vi "Event handler-Z Setup.vi"(8 "error in (no error)":errorcluster, 9 "Obtain Z Stop":bool, 11 "Obtain Z Start":bool) -> (0 "error out":errorcluster)   [LabVIEW 2020]
uses:
  Typedefs/Read Write Enum.ctl
  Global Variables/gl_UI Ctrl Refs.vi
  Global Variables/General Globals.vi
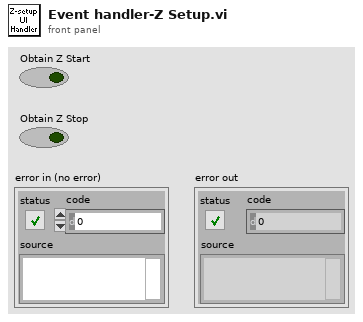
[diagram p1: front panel]
types:
  T1 = typedef "Read Write Enum.ctl" = enum16{"Read", "Write"}
  T2 = typedef "UI ctrl refs cluster.ctl" = cluster{"Top level VI path":path, "Top level VI ref":refnum<vi>, "User menu ref":refnum<k9>, "Sub Panel control":refnum<vi>, "Imaging Param Tab":refnum<vi>, "Occurrence-Start drivers":refnum<k4>, "Occurrence-Speed logging initialised":refnum<k4>, "Occurrence-XYZ stage initialised":refnum<k4>, "Exit button":refnum<vi>, "Status ind":refnum<vi>, "Set as origin":refnum<vi>, "Speed Logging":refnum<vi>, "Time Lapse":refnum<vi>, "Live Imaging":refnum<vi>, "AOL Z Stack":refnum<vi>, "Motor Z Stack":refnum<vi>, "Funct Acq button":refnum<vi>, "Hard Shutter":refnum<vi>, "Virtual Shutter":refnum<vi>, "Laser Power":refnum<vi>, "AOL Mode":refnum<vi>, "Frame Size":refnum<vi>, "Field of View":refnum<vi>, "Dwell Time":refnum<vi>, "Zoom":refnum<vi>, "AOL Z":refnum<vi>, "Objective":refnum<vi>, "Axis":refnum<vi>, "Paths & Names":refnum<vi>, "Experiment folder path (ind.)":refnum<vi>, "Last State (Ind.)":refnum<vi>, "Averages":refnum<vi>, "Angle (degrees)":refnum<vi>, "X centre":refnum<vi>, "Y centre":refnum<vi>, "Plane Mode":refnum<vi>, "# Planes":refnum<vi>, "Z Start":refnum<vi>, "Z Stop":refnum<vi>, "Z Step":refnum<vi>, "PMT 1":refnum<vi>, "PMT 2":refnum<vi>, "Stage XYZ Position":refnum<vi>, "Pockels@Z Start":refnum<vi>, "Pockels@Z Stop":refnum<vi>, "Obtain Z Start":refnum<vi>, "Obtain Z Stop":refnum<vi>, "Live stim.trig.period":refnum<vi>, "Live stim.trig.enable":refnum<vi>, "Movement Correction":refnum<vi>, "Load Reference Image":refnum<vi>, "XY Stage Move":refnum<vi>, "MovCor Cluster":refnum<vi>, "RefDAQParam":refnum<vi>, "Funct. Acq. Pockels Modulation":refnum<vi>, "Ref Laser Power":refnum<vi>, "Enable Video Recording":refnum<vi>, "Video Record-Live Imaging":refnum<vi>, "Video Record-Funct acq":refnum<vi>, "Reference Source":refnum<vi>, "AOL Z-stack Chirps Ready (ind)":refnum<vi>, "Target time between mov.cor. ref triggers (ms)":refnum<vi>, "Funct. Acq. Ref frame save":refnum<vi>, "Tracking button":refnum<vi>, "Show ref plots window":refnum<vi>, "Center freq ind (nm)":refnum<vi>, "Pickup mode (ind)":refnum<vi>, "Logging queue (ind)":refnum<vi>, "Back aperture power (ind.)":refnum<vi>, "Power after objective (ind.)":refnum<vi>, "Switch user":refnum<vi>, "Ls1 Conn. Status":refnum<vi>, "Ls1Tuning Status":refnum<vi>, "Ls1 Faults":refnum<vi>, "Ls1 Connection":refnum<vi>, "Ls1 Mode":refnum<vi>, "Ls1 POWER [mW]":refnum<vi>, "Ls1Shutter":refnum<vi>, "Ls1 Wavelength":refnum<vi>, "Ls1 Note":refnum<vi>, "Ls1 Confirm Wav":refnum<vi>, "Ls1 PreChrp Prism1":refnum<vi>, "Ls1 PreChrp Prism2":refnum<vi>, "Ls1 wav top Ind":refnum<vi>, "Ls1 power top Ind":refnum<vi>, "Ls1 Pump peak Hold":refnum<vi>, "Ls1 Status Ind":refnum<vi>, "Ls1 wav cancel":refnum<vi>, "Experiment Type":refnum<vi>, "Biology Information":refnum<vi>, "Camera recording status":refnum<vi>, "Parameter Sweep Steps":refnum<vi>, "Parameter Sweep":refnum<vi>, "Gen. Sweep Chirps":refnum<vi>, "Sweep Chirps ready":refnum<vi>, "# Sw. Planes":refnum<vi>, "Start Sweep":refnum<vi>, "Low-High Resolution Settings":refnum<vi>, "Optimise Obj. Pos.":refnum<vi>}
  T3 = typedef "Laser control knob.ctl" = u16
  T4 = cluster{"ZStack":cluster{"Zstart":dbl, "Zstop":dbl, "Zstep":dbl}, "Laser Power %":cluster{"@ Start":dbl, "@ Stop":dbl}}
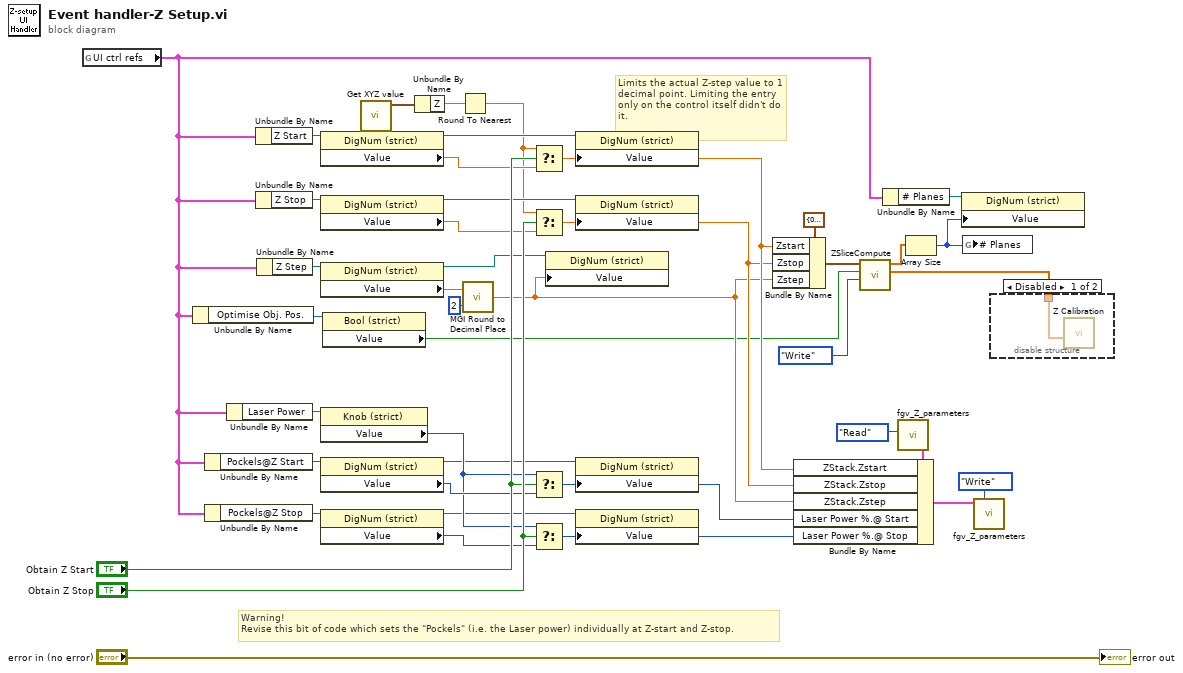
[diagram p0: block diagram]
diagram:
  # "Limits the actual Z-step value to 1 decimal point. Limiting the entry only on the control itself didn't do it."
  # "Warning!\nRevise this bit of code which sets the \"Pockels\" (i.e. the Laser power) individually at Z-start and Z-stop."
  n1 = global read "gl_UI Ctrl Refs.vi" "UI ctrl refs"() -> (w2:T2)
  n2 = Unbundle By Name(w2) -> ("Optimise Obj. Pos."=w3:refnum<vi>)
  n3 = Unbundle By Name(w2) -> ("Pockels@Z Start"=w19:refnum<vi>)
  n4 = Unbundle By Name(w2) -> ("Pockels@Z Stop"=w18:refnum<vi>)
  n5 = Unbundle By Name(w2) -> ("Laser Power"=w20:refnum<vi>)
  n6 = Unbundle By Name(w2) -> ("Z Start"=w26:refnum<vi>)
  n7 = Unbundle By Name(w2) -> ("Z Stop"=w25:refnum<vi>)
  n8 = Unbundle By Name(w2) -> ("Z Step"=w21:refnum<vi>)
  n9 = property on="Property Node" class="DigNum (strict)"(reference=w26) -> (reference out=w29:refnum<vi>, "Value"=w28:dbl)  [unwired: 1 in, 1 out]
  n10 = property on="Property Node" class="DigNum (strict)"(reference=w25) -> (reference out=w24:refnum<vi>, "Value"=w23:dbl)  [unwired: 1 in, 1 out]
  n11 = property on="Property Node" class="DigNum (strict)"(reference=w21) -> (reference out=w5:refnum<vi>, "Value"=w6:dbl)  [unwired: 1 in, 1 out]
  n12 = property on="Property Node" class="Knob (strict)"(reference=w20) -> ("Value"=w35:T3)  [unwired: 1 in, 2 out]
  n13 = property on="Property Node" class="DigNum (strict)"(reference=w19) -> (reference out=w17:refnum<vi>, "Value"=w36:u16)  [unwired: 1 in, 1 out]
  n14 = property on="Property Node" class="DigNum (strict)"(reference=w18) -> (reference out=w16:refnum<vi>, "Value"=w34:u16)  [unwired: 1 in, 1 out]
  n15 = property on="Property Node" class="Bool (strict)"(reference=w3) -> ("Value"=w1:bool)  [unwired: 1 in, 2 out]
  n16 = call "Get XYZ value.vi"() -> ("Stage XYZ Position"=w10:cluster{"X":sgl, "Y":sgl, "Z":sgl})  [unwired: 11 in]
  n17 = Unbundle By Name(w10) -> ("Z"=w37:sgl)
  n18 = Round To Nearest(number=w37) -> (nearest integer value=w8:sgl)
  n19 = call <userlib>:"MGI Round to Decimal Place.vi"("Decimal Digits"=2, "Number"=w6) -> ("Rounded"=w4:dbl)  [unwired: 1 in]
  n20 = Select(t=w8, s="Obtain Z Start", f=w28) -> (s? t:f=w27:dbl)
  n21 = Select(t=w8, s="Obtain Z Stop", f=w23) -> (s? t:f=w22:dbl)
  n22 = Select(t=w35, s="Obtain Z Start", f=w36) -> (s? t:f=w15:T3)
  n23 = Select(t=w35, s="Obtain Z Stop", f=w34) -> (s? t:f=w14:T3)
  n24 = property on="Property Node" class="DigNum (strict)"(reference=w5, "Value"=w4) -> ()  [unwired: 1 in, 2 out]
  n25 = property on="Property Node" class="DigNum (strict)"(reference=w29, "Value"=w27) -> ()  [unwired: 1 in, 2 out]
  n26 = property on="Property Node" class="DigNum (strict)"(reference=w24, "Value"=w22) -> ()  [unwired: 1 in, 2 out]
  n27 = property on="Property Node" class="DigNum (strict)"(reference=w17, "Value"=w15) -> ()  [unwired: 1 in, 2 out]
  n28 = property on="Property Node" class="DigNum (strict)"(reference=w16, "Value"=w14) -> ()  [unwired: 1 in, 2 out]
  n29 = Bundle By Name(cluster=cluster{"Zstart":dbl, "Zstop":dbl, "Zstep":dbl} {"Zstart"=0.0, "Zstop"=0.0, "Zstep"=0.0} ("ZStack"), "Zstart"=w27, "Zstop"=w22, "Zstep"=w4) -> (w40:cluster{"Zstart":dbl, "Zstop":dbl, "Zstep":dbl})
  n30 = call "ZSliceCompute.vi"("Function"=Read_Write_Enum."Write", "Optimise Objective position"=w1, "ZStack (um)"=w40) -> ("AOL Z Planes(um)"=w38:dbl[], "Motor Z Planes(um)"=w39:dbl[])  [unwired: 5 in, 2 out]
  n31 = Unbundle By Name(w2) -> ("# Planes"=w13:refnum<vi>)
  n32 = call "fgv_Z_parameters.vi"("Function"=enum16{"Intialize", "Write", "Read", "Clear"}."Read") -> ("Z Parameters"=w31:T4)  [unwired: 9 in, 1 out]
  n33 = Bundle By Name(cluster=w31, "ZStack.Zstart"=w27, "ZStack.Zstop"=w22, "ZStack.Zstep"=w4, "Laser Power %.@ Start"=w15, "Laser Power %.@ Stop"=w14) -> (w30:T4)
  n34 = Array Size(array=w39) -> (size(s)=w11:i32)
  n35 = property on="Property Node" class="DigNum (strict)"(reference=w13, "Value"=w11) -> ()  [unwired: 1 in, 2 out]
  n36 = global write "General Globals.vi" "# Planes"(w11) -> ()
  n37 = call "fgv_Z_parameters.vi"("Function"=enum16{"Intialize", "Write", "Read", "Clear"}."Write", "Z Parameters"=w30) -> ()  [unwired: 8 in, 2 out]
  n38 = disable-structure "Diagram Disable Structure" shown="Disabled" {
    disable-tunnel: w38 -> [w44 _]
    frame Disabled {
      n39 = call "Z Calibration.vi"("Z Planes"=w44) -> ()  [unwired: 7 in, 4 out]
    }
    frame Enabled {
    }
  }
  "error out" <- "error in (no error)"
